vi "log-all-data.vi"(0 "log-file-byte-stream":refnum<file>, 1 "CSV Data Headings":string, 2 "adam5000:all-data-in":T3, 3 "log-start-time(mS)":u32, 4 "file open?":bool, 5 "error in (no error)":errorcluster, 6 "Log Filepath Selection":T2, 7 "Start Logging":bool) -> (10 "appended path for log file":path, 11 "log-elapsed time":dbl format="%.2f", 12 "log-filepath-enable-state":T1(ring), 13 "Start Logging":bool, 14 "log-file-bytestream":refnum<file>, 15 "Logged Data String":string, 17 "log-start-time(mS)":u32, 18 "file open?":bool, 19 "error out":errorcluster)   [LabVIEW 2024]
uses:
  controls/adam-5000-all-chassis-data.ctl
  controls/adam-5000-all-module-datas.ctl
  controls/digital-output-cluster.ctl
  controls/digitial-input-cluster.ctl
  controls/analog-output-cluster.ctl
  controls/analog-input-cluster.ctl
  controls/thermocouple-input-cluster.ctl
  csv-file-logging/filepath-selection.ctl
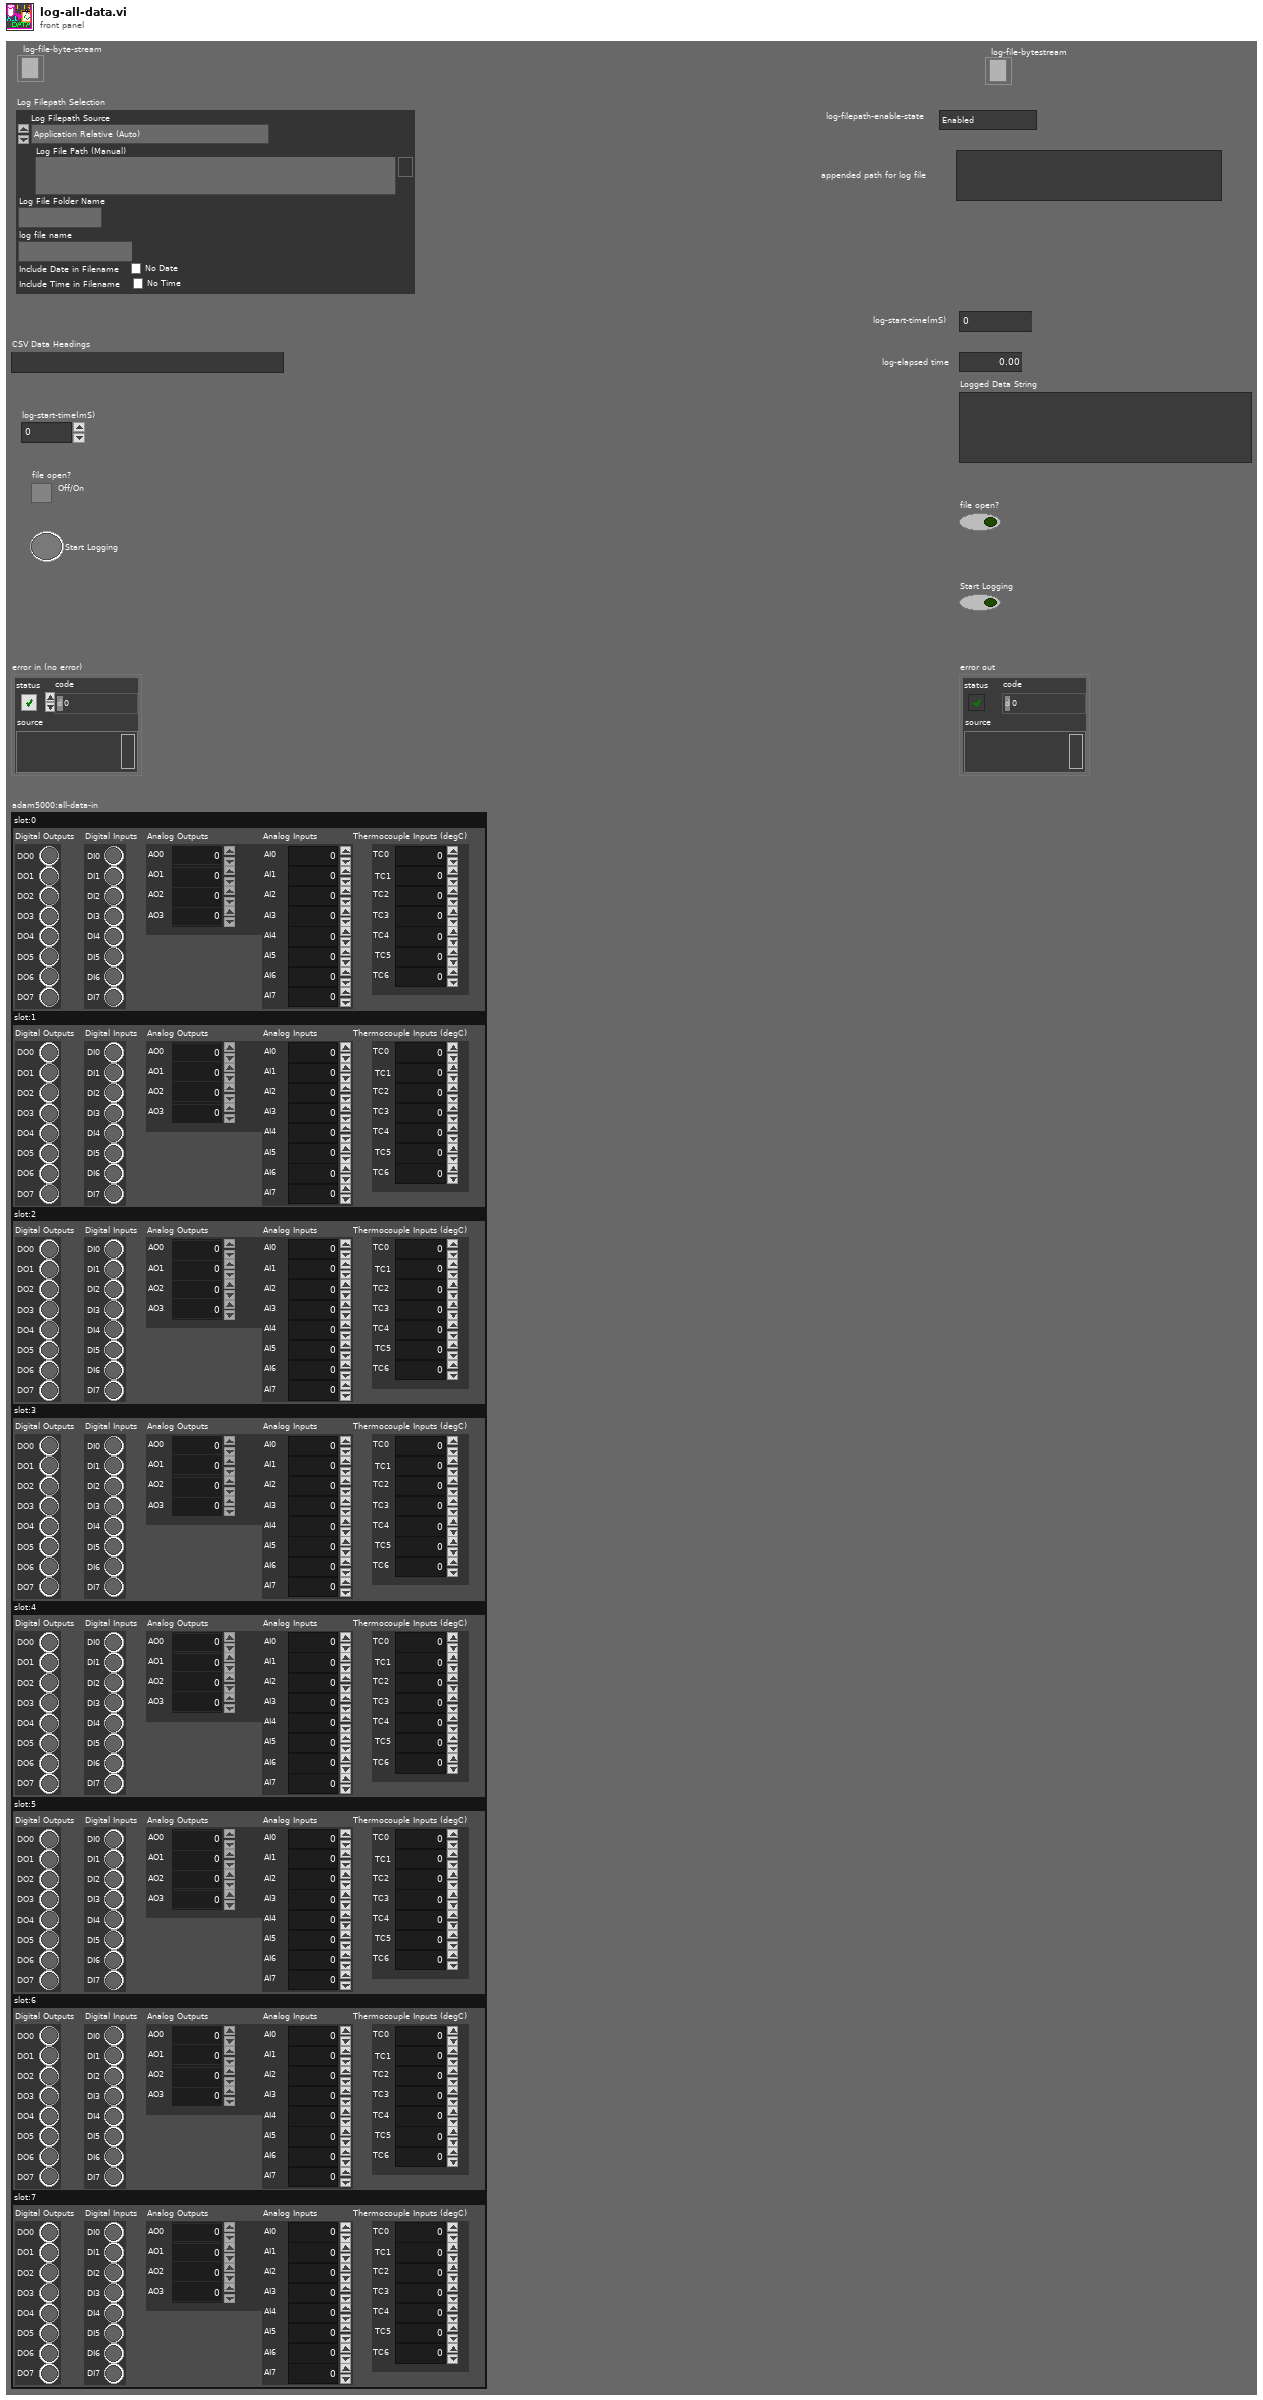
[diagram p1: front panel]
types:
  T1 = enum8{"Enabled", "Disabled", "Disabled and Grayed Out"}
  T2 = typedef "filepath-selection.ctl" = cluster{"Log Filepath Source":enum16{"Application Relative (Auto)", "VI Relative (Auto)", "Complete Path (Manual)"}, "Log File Path (Manual)":path, "Log File Folder Name":string, "log file name":string, "Include Date in Filename":bool, "Include Time in Filename":bool}
  T3 = typedef "adam-5000-all-chassis-data.ctl" = cluster{"slot:0":T4, "slot:1":T4, "slot:2":T4, "slot:3":T4, "slot:4":T4, "slot:5":T4, "slot:6":T4, "slot:7":T4}
  T4 = typedef "adam-5000-all-module-datas.ctl" = cluster{"Digital Outputs":T5, "Digital Inputs":T6, "Analog Outputs":T7, "Analog Inputs":T8, "Thermocouple Inputs (degC)":T9}
  T5 = typedef "digital-output-cluster.ctl" = cluster{"DO0":bool, "DO1":bool, "DO2":bool, "DO3":bool, "DO4":bool, "DO5":bool, "DO6":bool, "DO7":bool}
  T6 = typedef "digitial-input-cluster.ctl" = cluster{"DI0":bool, "DI1":bool, "DI2":bool, "DI3":bool, "DI4":bool, "DI5":bool, "DI6":bool, "DI7":bool}
  T7 = typedef "analog-output-cluster.ctl" = cluster{"AO0":dbl, "AO1":dbl, "AO2":dbl, "AO3":dbl}
  T8 = typedef "analog-input-cluster.ctl" = cluster{"AI0":dbl, "AI1":dbl, "AI2":dbl, "AI3":dbl, "AI4":dbl, "AI5":dbl, "AI6":dbl, "AI7":dbl}
  T9 = typedef "thermocouple-input-cluster.ctl" = cluster{"TC0":dbl, "TC1":dbl, "TC2":dbl, "TC3":dbl, "TC4":dbl, "TC5":dbl, "TC6":dbl}
  T10 = enum16{"open", "replace", "create", "open or create", "replace or create", "replace or create with confirmation"}
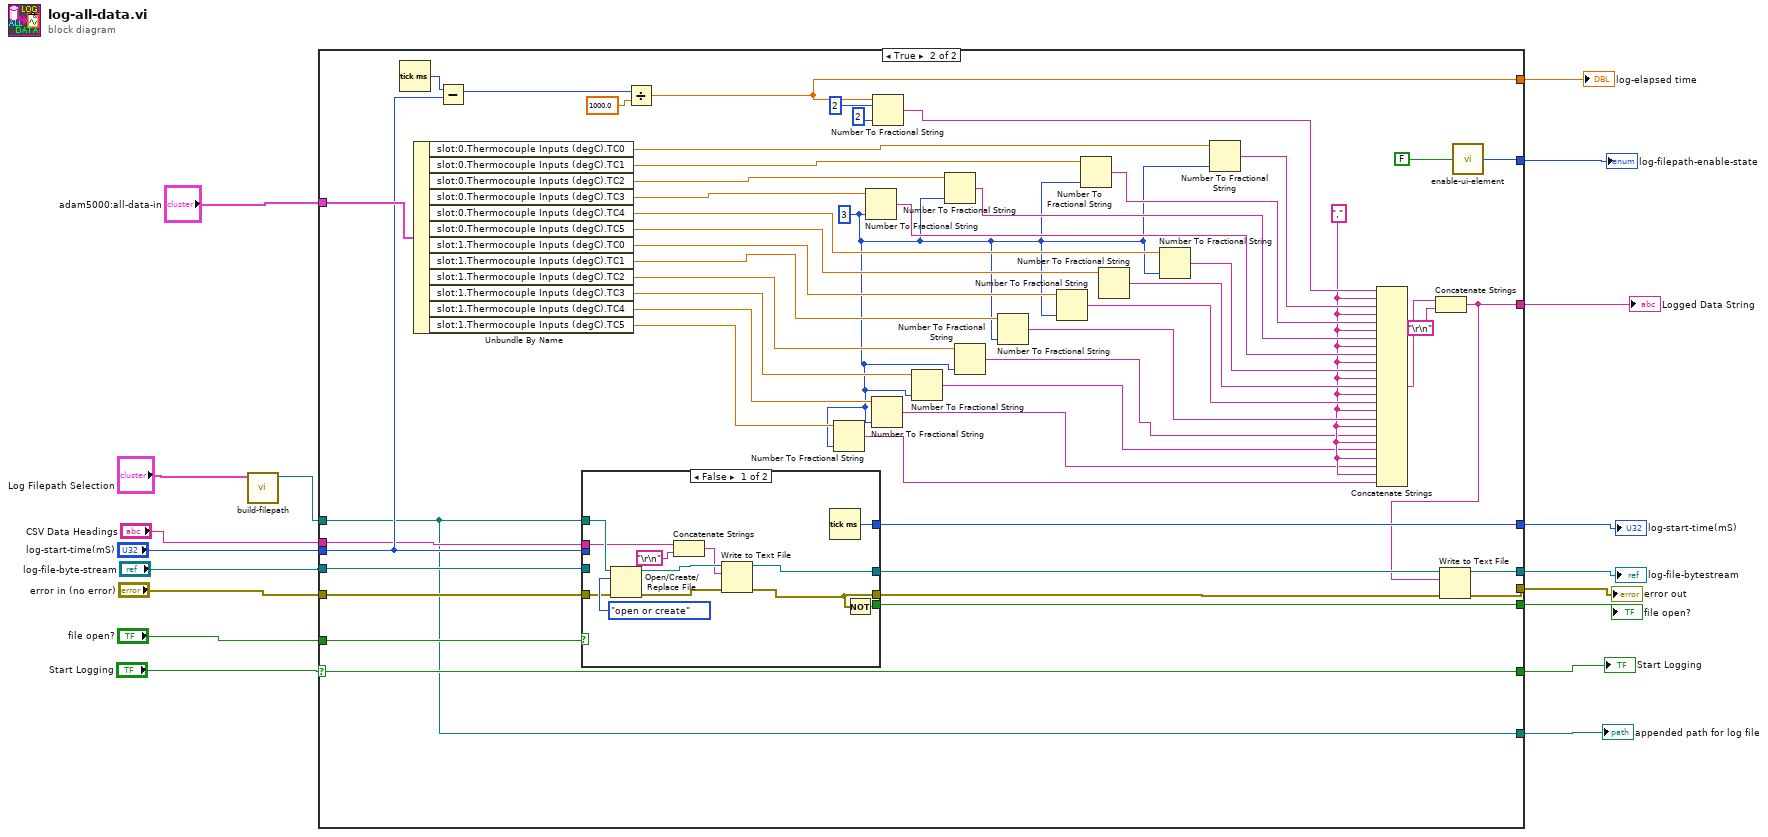
[diagram p0: block diagram]
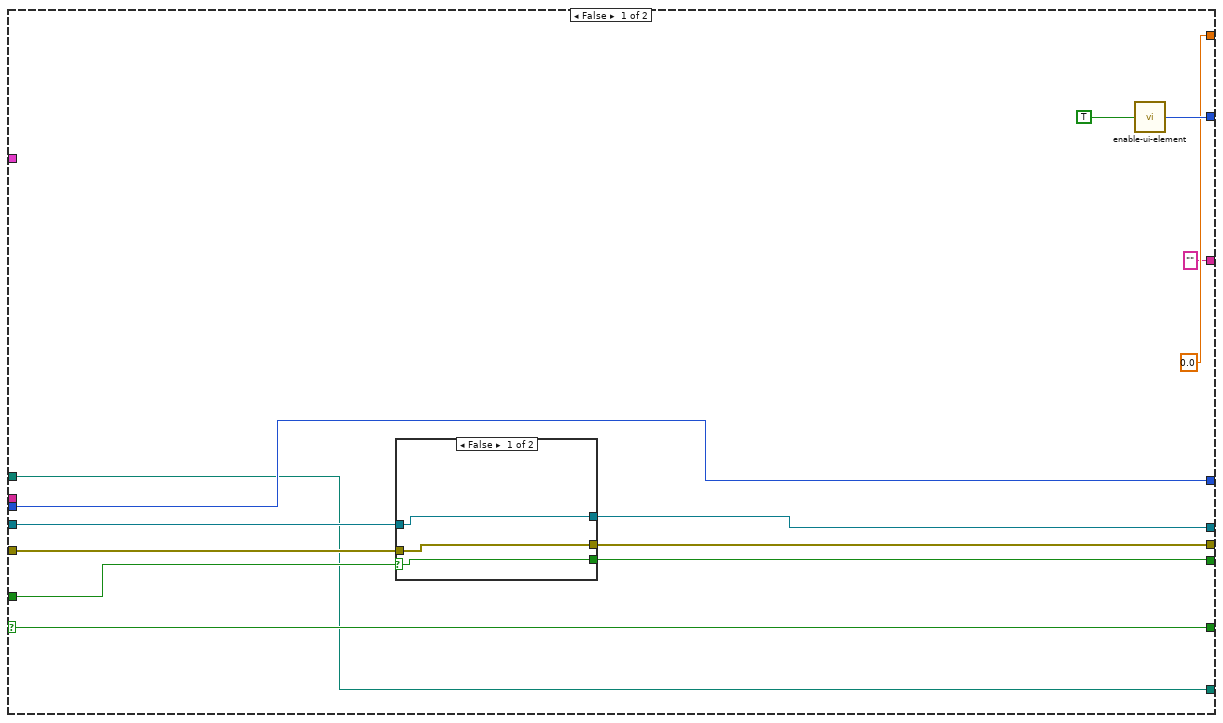
[diagram p2: hidden frame]
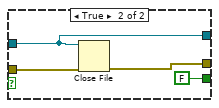
[diagram p3: hidden frame]
diagram:
  n1 = call "build-filepath.vi"("Log Filepath Selection"="Log Filepath Selection") -> ("appended path for log file"=w10:path)  [unwired: 9 in, 1 out]
  n2 = case shown="True" "Start Logging" {
    selector: "Start Logging" -> [w31 w87]
    tunnel: [w31 w87] -> w7
    tunnel: [w22 w88] -> w8
    tunnel: w10 -> [w21 w66]
    tunnel: "adam5000:all-data-in" -> [_ w90]
    tunnel: [w29 w84] -> w12
    tunnel: "file open?" -> [w30 w86]
    tunnel: "error in (no error)" -> [w27 w85]
    tunnel: [w26 w74] -> w14
    tunnel: [w25 w76] -> w15
    tunnel: "log-file-byte-stream" -> [w28 w83]
    tunnel: [w24 w82] -> w17
    tunnel: "log-start-time(mS)" -> [w24 w80]
    tunnel: "CSV Data Headings" -> [_ w78]
    tunnel: ["" w54] -> w3
    tunnel: [0.0 w67] -> w2
    tunnel: [w21 w66] -> w1
    frame False {
      n3 = case shown="False" w30 {
        selector: w30 -> [w32 _]
        tunnel: [w32 FALSE] -> w29
        tunnel: w28 -> [w34 w35]
        tunnel: w27 -> [w33 w37]
        tunnel: [w33 w36] -> w26
        tunnel: [w34 w35] -> w25
        frame False {
        }
        frame True {
          n4 = Close File(refnum=w35, error in=w37) -> (error out=w36:errorcluster)  [unwired: 1 out]
        }
      }
      n5 = call "enable-ui-element.vi"("Enable UI Element"=TRUE) -> ("UI Element State"=w22:T1)  [unwired: 8 in]
    }
    frame True {
      w43 = "," ("string")
      w45 = i16 3 ("precision (6)")
      n6 = Tick Count (ms)() -> (millisecond timer value=w81:u32)
      n7 = Unbundle By Name(w90) -> ("slot:0.Thermocouple Inputs (degC).TC0"=w73:dbl, "slot:0.Thermocouple Inputs (degC).TC1"=w70:dbl, "slot:0.Thermocouple Inputs (degC).TC2"=w69:dbl, "slot:0.Thermocouple Inputs (degC).TC3"=w72:dbl, "slot:0.Thermocouple Inputs (degC).TC4"=w53:dbl, "slot:0.Thermocouple Inputs (degC).TC5"=w52:dbl, "slot:1.Thermocouple Inputs (degC).TC0"=w51:dbl, "slot:1.Thermocouple Inputs (degC).TC1"=w50:dbl, "slot:1.Thermocouple Inputs (degC).TC2"=w49:dbl, "slot:1.Thermocouple Inputs (degC).TC3"=w48:dbl, "slot:1.Thermocouple Inputs (degC).TC4"=w47:dbl, "slot:1.Thermocouple Inputs (degC).TC5"=w46:dbl)
      n8 = Subtract(x=w81, y=w80) -> (x-y=w79:u32)
      n9 = case shown="False" w86 {
        selector: w86 -> [_ w106]
        tunnel: w66 -> [w101 _]
        tunnel: w85 -> [w100 w105]
        tunnel: [w95 w105] -> w75
        tunnel: [w99 w106] -> w84
        tunnel: [w94 w103] -> w77
        tunnel: w83 -> [_ w103]
        tunnel: [w98 w104] -> w82
        tunnel: w80 -> [_ w104]
        tunnel: w78 -> [w92 _]
        frame False {
          n10 = Open/Create/Replace File(file path (use dialog)=w101, error in=w100, operation (0:open)=T10."open or create") -> (refnum out=w97:refnum<file>, error out=w96:errorcluster)  [unwired: 3 in, 1 out]
          n11 = Concatenate Strings(w92, "\r\n") -> (w91:string)
          n12 = Write to Text File(file (use dialog)=w97, text=w91, error in=w96) -> (refnum out=w94:refnum<file>, error out=w95:errorcluster)  [unwired: 1 in, 1 out]
          n13 = Tick Count (ms)() -> (millisecond timer value=w98:u32)
          n14 = Not(x=w95) -> (.not. x?=w99:bool)
        }
        frame True {
        }
      }
      n15 = Divide(x=w79, y=1000.0) -> (x/y=w67:dbl)
      n16 = Number To Fractional String(number=w46, precision (6)=w45) -> (F-format string=w39:string)  [unwired: 2 in]
      n17 = Number To Fractional String(number=w72, precision (6)=w45) -> (F-format string=w58:string)  [unwired: 2 in]
      n18 = Number To Fractional String(number=w47, precision (6)=w45) -> (F-format string=w40:string)  [unwired: 2 in]
      n19 = Number To Fractional String(number=w67, width (-)=i16 2, precision (6)=i16 2) -> (F-format string=w65:string)  [unwired: 1 in]
      n20 = Number To Fractional String(number=w48, precision (6)=w45) -> (F-format string=w41:string)  [unwired: 2 in]
      n21 = Number To Fractional String(number=w69, precision (6)=w45) -> (F-format string=w59:string)  [unwired: 2 in]
      n22 = Number To Fractional String(number=w49, precision (6)=w45) -> (F-format string=w42:string)  [unwired: 2 in]
      n23 = Number To Fractional String(number=w50, precision (6)=w45) -> (F-format string=w44:string)  [unwired: 2 in]
      n24 = Number To Fractional String(number=w51, precision (6)=w45) -> (F-format string=w55:string)  [unwired: 2 in]
      n25 = Number To Fractional String(number=w70, precision (6)=w45) -> (F-format string=w60:string)  [unwired: 2 in]
      n26 = Number To Fractional String(number=w52) -> (F-format string=w56:string)  [unwired: 3 in]
      n27 = Number To Fractional String(number=w53, precision (6)=w45) -> (F-format string=w57:string)  [unwired: 2 in]
      n28 = Number To Fractional String(number=w73, precision (6)=w45) -> (F-format string=w61:string)  [unwired: 2 in]
      n29 = Concatenate Strings(w65, w43, w61, w43, w60, w43, w59, w43, w58, w43, w57, w43, w56, w43, w55, w43, w44, w43, w42, w43, w41, w43, w40, w43, w39) -> (w63:string)
      n30 = Concatenate Strings(w63, "\r\n") -> (w54:string)
      n31 = Write to Text File(file (use dialog)=w77, text=w54, error in=w75) -> (refnum out=w76:refnum<file>, error out=w74:errorcluster)  [unwired: 1 in, 1 out]
      n32 = call "enable-ui-element.vi"("Enable UI Element"=FALSE) -> ("UI Element State"=w88:T1)  [unwired: 8 in]
    }
  }
  "log-start-time(mS)" <- w17
  "log-file-bytestream" <- w15
  "error out" <- w14
  "file open?" <- w12
  "appended path for log file" <- w1
  "log-filepath-enable-state" <- w8
  "Start Logging" <- w7
  "Logged Data String" <- w3
  "log-elapsed time" <- w2
